vi "GOOP_VI_Provider_OnPopupMenu.vi"(11 "objects":T1[](array[typedef])) -> ()   [LabVIEW 2020]
uses:
  <resource>/Framework/Providers/API/ItemRef.ctl
  <resource>/Framework/Providers/API/mxLvMenuItem.ctl
panel:
  out "error out":errorcluster
  in  "error in":errorcluster
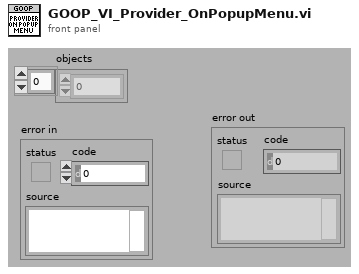
[diagram p1: front panel]
types:
  T1 = typedef "ItemRef.ctl" = u64
  T2 = typedef "mxLvMenuItem.ctl" = cluster{"Menu Name":string, "Description":string, "Icon File Name":path, "Menu Tag":string, "Enabled":bool, "Checked":bool, "Separator":bool, "Batchable":bool, "Weight":i32, "Batch Mode (Ignored if Not Batchable)":enum32{"Show If All Items Support Command", "Show If Any Items Support Command"}, "Menu Location":enum32{"<None>", "Project", "Project / Build Specifications", "Tools", "Tools / Source Control", "Tools / Real-Time Module", "Help"}, "Exclude From Getting Started Window Menu":bool}
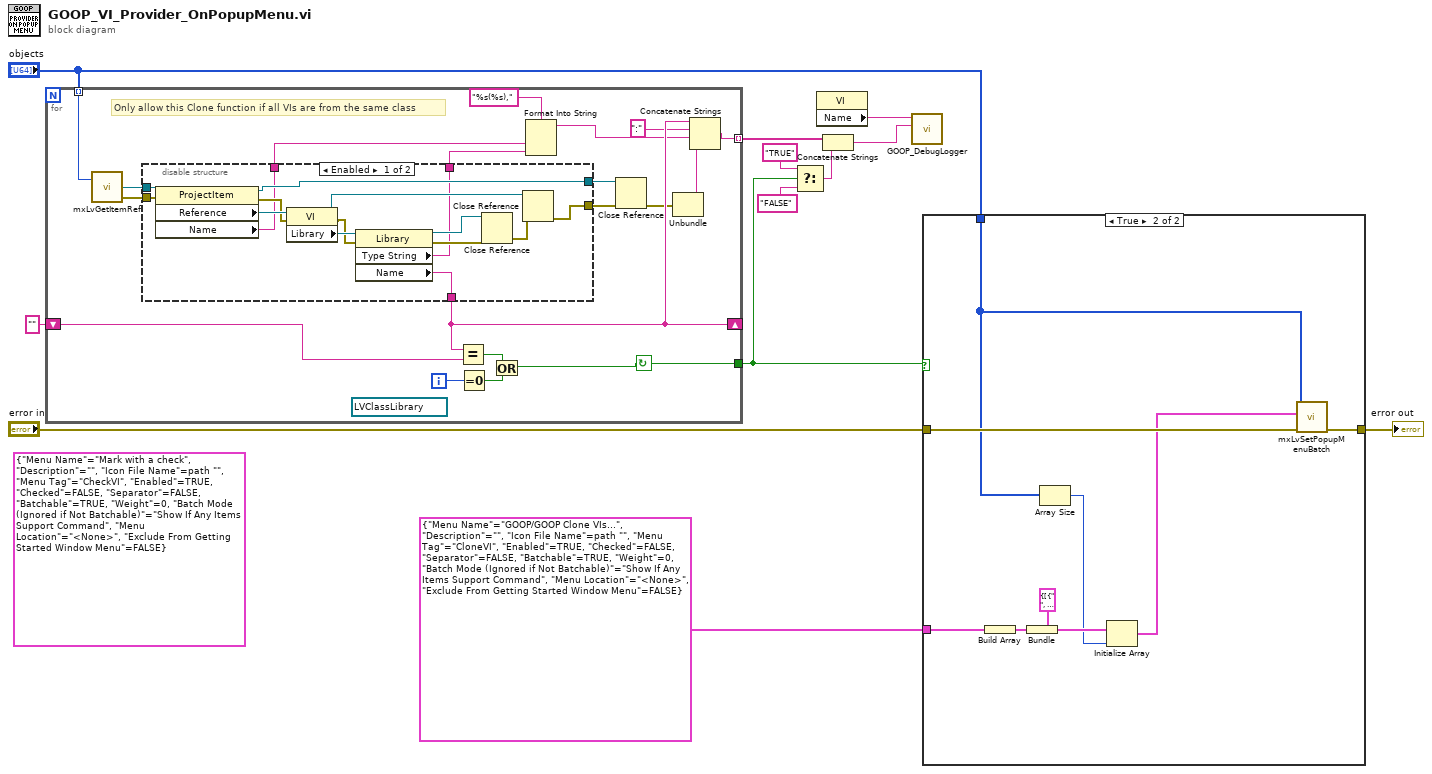
[diagram p0: block diagram]
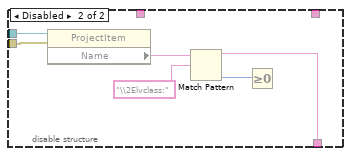
[diagram p3: hidden frame]
diagram:
  (unwired) T2 {"Menu Name"="Mark with a check", "Description"="", "Icon File Name"=path "", "Menu Tag"="CheckVI", "Enabled"=TRUE, "Checked"=FALSE, "Separator"=FALSE, "Batchable"=TRUE, "Weight"=0, "Batch Mode (Ignored if Not Batchable)"=enum."Show If Any Items Support Command", "Menu Location"=enum."<None>", "Exclude From Getting Started Window Menu"=FALSE} ("Menu Item")
  n1 = for {
    tunnel: "objects" -> [w31] mode=indexing
    shift-right: [w23] -> _
    shift-left: "" ("Name") -> [w27]
    tunnel: [w17] -> w4
    tunnel: [w22] -> w6 mode=indexing
    i -> [w26]
    stop <- w17 continue-if-true
    (unwired) refnum<vi> refnum ("Library")
    # "Only allow this Clone function if all VIs are from the same class"
    n2 = call <resource>:"mxLvGetItemRef.vi"("Item"=w31) -> ("Item Refnum"=w30:refnum<vi>, "error out"=w18:errorcluster)  [unwired: 1 in, 1 out]
    n3 = disable-structure shown="Enabled" {
      disable-tunnel: w30 -> [w46 w52]
      disable-tunnel: [w39 _] -> w29
      disable-tunnel: [w38 _] -> w28
      disable-tunnel: [w32 _] -> w15
      disable-tunnel: [w37 w48] -> w23
      disable-tunnel: w18 -> [w34 w51]
      disable-tunnel: [w33 _] -> w14
      frame Enabled {
        n4 = property class="ProjectItem"(reference=w46, error in=w34) -> (reference out=w38:refnum<vi>, error out=w35:errorcluster, "Reference"=w45:refnum<vi>, "Name"=w32:string)
        n5 = property class="VI"(reference=w45, error in=w35) -> (reference out=w41:refnum<vi>, error out=w36:errorcluster, "Library"=w44:refnum<vi>)
        n6 = property class="Library"(reference=w44, error in=w36) -> (reference out=w42:refnum<vi>, error out=w43:errorcluster, "Type String"=w33:string, "Name"=w37:string)
        n7 = Close Reference(reference=w42, error in (no error)=w43) -> (error out=w40:errorcluster)
        n8 = Close Reference(reference=w41, error in (no error)=w40) -> (error out=w39:errorcluster)
      }
      frame Disabled {
        n9 = property class="ProjectItem"(reference=w52, error in=w51) -> ("Name"=w50:string)  [unwired: 2 out]
        n10 = Match Pattern(string=w50, regular expression="\\2Elvclass:") -> (before substring=w48:string, offset past match=w47:i32)  [unwired: 1 in, 2 out]
        n11 = Greater Or Equal To 0?(x=w47) -> ()  [unwired: 1 out]
      }
    }
    n12 = Equal?(x=w23, y=w27) -> (x = y?=w25:bool)
    n13 = Equal To 0?(x=w26) -> (x = 0?=w24:bool)
    n14 = Or(x=w25, y=w24) -> (x .or. y?=w17:bool)
    n15 = Format Into String(format string="%s(%s),", w15, w14) -> (resulting string=w13:string)  [unwired: 2 in, 1 out]
    n16 = Close Reference(reference=w28, error in (no error)=w29) -> (error out=w20:errorcluster)
    n17 = Unbundle(w20) -> ("source"=w19:string)  [unwired: 2 out]
    n18 = Concatenate Strings(w23, ":", w13, w19) -> (w22:string)
  }
  n19 = Select(t="TRUE" ("Name"), s=w4, f="FALSE" ("Name")) -> (s? t:f=w2:string)
  n20 = property class="VI"() -> ("Name"=w7:string)  [unwired: 2 in, 2 out]
  n21 = Concatenate Strings(w6, w2) -> (w5:string)
  n22 = call <resource>:"GOOP_DebugLogger.vi"("Data"=w5, "State"=w7) -> ()  [unwired: 7 in, 3 out]
  n23 = case shown="True" w4 {
    tunnel: [w53 w62] -> w12
    tunnel: "error in" -> [w53 w61]
    tunnel: T2 {"Menu Name"="GOOP/GOOP Clone VIs...", "Description"="", "Icon File Name"=path "", "Menu Tag"="CloneVI", "Enabled"=TRUE, "Checked"=FALSE, "Separator"=FALSE, "Batchable"=TRUE, "Weight"=0, "Batch Mode (Ignored if Not Batchable)"=enum."Show If Any Items Support Command", "Menu Location"=enum."<None>", "Exclude From Getting Started Window Menu"=FALSE} ("Menu Item") -> [_ w59]
    tunnel: "objects" -> [_ w55]
    frame False {
    }
    frame True {
      n24 = Build Array(w59) -> (w58:T2[])
      n25 = Bundle(cluster=cluster{"Popup Menu Items":T2[]} {"Popup Menu Items"=[{"Menu Name"="", "Description"="", "Icon File Name"=path "", "Menu Tag"="", "Enabled"=TRUE, "Checked"=FALSE, "Separator"=FALSE, "Batchable"=TRUE, "Weight"=0, "Batch Mode (Ignored if Not Batchable)"=enum."Show If Any Items Support Command", "Menu Location"=enum."<None>", "Exclude From Getting Started Window Menu"=FALSE}]}, "Popup Menu Items"=w58) -> (w57:cluster{"Popup Menu Items":T2[]})
      n26 = Array Size(array=w55) -> (size(s)=w56:i32)
      n27 = Initialize Array(w57, w56) -> (w54:cluster{"Popup Menu Items":T2[]}[])
      n28 = call <resource>:"mxLvSetPopupMenuBatch.vi"("error in"=w61, "Menu Items"=w54, "Items"=w55) -> ("error out"=w62:errorcluster)  [unwired: 7 in, 1 out]
    }
  }
  "error out" <- w12
